vi "ReshapeItemArray.vi"(11 "Array":refnum<class "Link.lvclass">[](array[class])) -> (1 "ring info":refnum<class "RingItem.lvclass">[](array[class]), 3 "item info array":T1(array[cluster]))   [LabVIEW 2023, in "GettingStartedWindow.lvlib"]
uses:
  <resource>/modes/FRC/GettingStartedWindow.lvlib
  <resource>/modes/FRC/Classes/Link/Link.lvclass
  <resource>/modes/FRC/Classes/ClickableText/ClickableText.lvclass
  <resource>/modes/FRC/Classes/RingItem/RingItem.lvclass
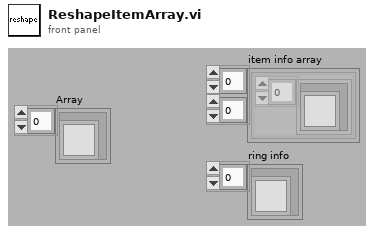
[diagram p1: front panel]
types:
  T1 = cluster{refnum<class "ClickableText.lvclass">[]}[][]
  T2 = typedef "GettingStartedWindow.lvlib/PositionCategory.ctl" = enum16{"none", "column 1", "column 2", "ring"}
  T3 = cluster{refnum<class "ClickableText.lvclass">[]}[]
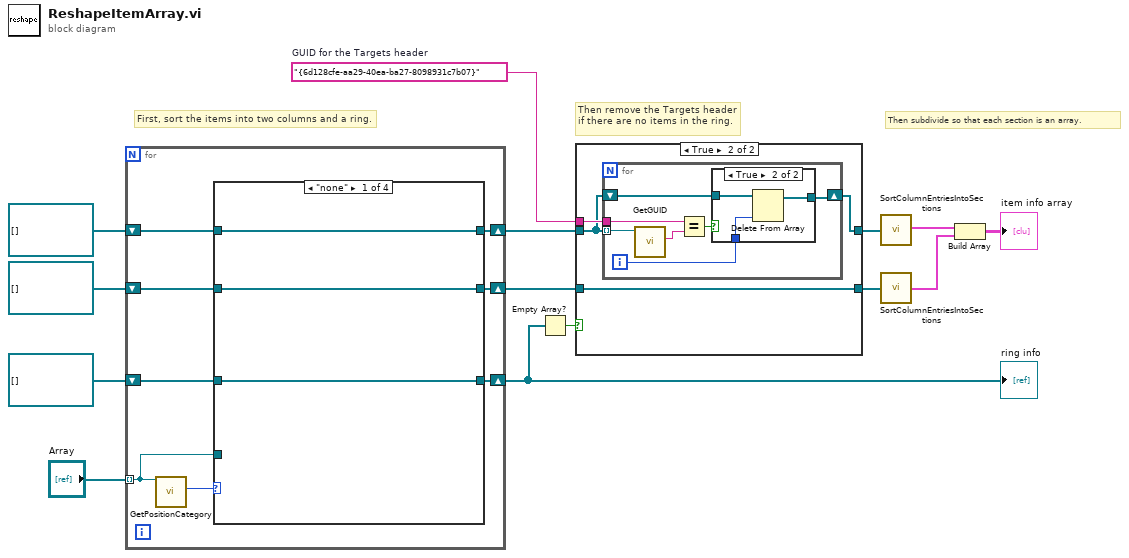
[diagram p0: block diagram]
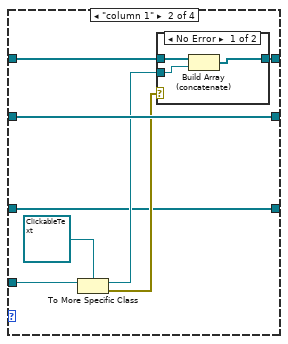
[diagram p4: hidden frame]
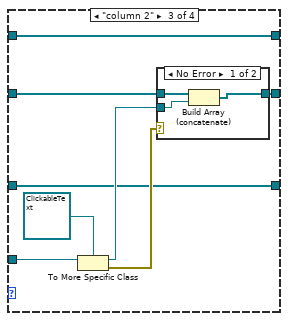
[diagram p6: hidden frame]
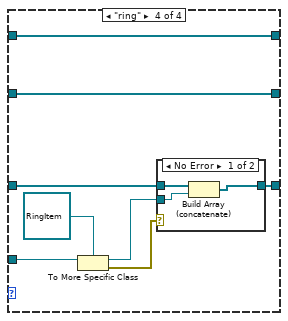
[diagram p8: hidden frame]
diagram:
  w1 = "{6d128cfe-aa29-40ea-ba27-8098931c7b07}"  # GUID for the Targets header
  # "Then remove the Targets header\nif there are no items in the ring."
  # "Then subdivide so that each section is an array."
  # "First, sort the items into two columns and a ring."
  n1 = for {
    tunnel: "Array" -> [w17] mode=indexing
    shift-right: [w20] -> w5
    shift-left: refnum<class "ClickableText.lvclass">[] [] -> [w21]
    shift-right: [w18] -> w3
    shift-left: refnum<class "ClickableText.lvclass">[] [] -> [w19]
    shift-right: [w15] -> w7
    shift-left: refnum<class "RingItem.lvclass">[] [] -> [w16]
    n2 = call-dynamic "GetPositionCategory.vi"("Link in"=w17) -> ("position"=w22:T2)  [unwired: 8 in, 2 out]
    n3 = case shown="\"none\"" w22 {
      tunnel: w21 -> [w25 w33 w40 w53]
      tunnel: w17 -> [_ w30 w45 w57]
      tunnel: [w25 w32 w40 w53] -> w20
      tunnel: w19 -> [w24 w31 w41 w52]
      tunnel: [w24 w31 w39 w52] -> w18
      tunnel: w16 -> [w23 w26 w38 w51]
      tunnel: [w23 w26 w38 w50] -> w15
      frame "none" {
      }
      frame "column 1" {
        n4 = To More Specific Class(target class=refnum<class "ClickableText.lvclass"> refnum ("GettingStartedWindow.lvlib:ClickableText.lvclass"), reference=w30) -> (specific class reference=w28:refnum<class "ClickableText.lvclass">, error out=w27:errorcluster)  [unwired: 1 in]
        n5 = case shown="No Error" w27 {
          tunnel: w33 -> [w36 w37]
          tunnel: [w35 w37] -> w32
          tunnel: w28 -> [w34 _]
          frame No Error {
            n6 = Build Array (concatenate)(w36, w34) -> (w35:refnum<class "ClickableText.lvclass">[])
          }
          frame Error {
          }
        }
      }
      frame "column 2" {
        n7 = To More Specific Class(target class=refnum<class "ClickableText.lvclass"> refnum ("GettingStartedWindow.lvlib:ClickableText.lvclass"), reference=w45) -> (specific class reference=w43:refnum<class "ClickableText.lvclass">, error out=w42:errorcluster)  [unwired: 1 in]
        n8 = case shown="No Error" w42 {
          tunnel: w41 -> [w48 w49]
          tunnel: [w47 w49] -> w39
          tunnel: w43 -> [w46 _]
          frame No Error {
            n9 = Build Array (concatenate)(w48, w46) -> (w47:refnum<class "ClickableText.lvclass">[])
          }
          frame Error {
          }
        }
      }
      frame "ring" {
        n10 = To More Specific Class(target class=refnum<class "RingItem.lvclass"> refnum ("GettingStartedWindow.lvlib:RingItem.lvclass"), reference=w57) -> (specific class reference=w55:refnum<class "RingItem.lvclass">, error out=w54:errorcluster)  [unwired: 1 in]
        n11 = case shown="No Error" w54 {
          tunnel: w51 -> [w60 w61]
          tunnel: [w59 w61] -> w50
          tunnel: w55 -> [w58 _]
          frame No Error {
            n12 = Build Array (concatenate)(w60, w58) -> (w59:refnum<class "RingItem.lvclass">[])
          }
          frame Error {
          }
        }
      }
    }
  }
  "ring info" <- w7
  n13 = Empty Array?(array=w7) -> (empty?=w6:bool)
  n14 = case shown="True" w6 {
    tunnel: w5 -> [w63 w65]
    tunnel: [w63 w64] -> w4
    tunnel: [w62 w67] -> w2
    tunnel: w3 -> [w62 w67]
    tunnel: w1 -> [_ w66]
    frame False {
    }
    frame True {
      n15 = for {
        tunnel: w65 -> [w74] mode=indexing
        tunnel: w66 -> [w72]
        shift-right: [w68] -> w64
        shift-left: w65 -> [w70]
        i -> [w69]
        n16 = call <resource>:"GetGUID.vi"("Link in"=w74) -> ("GUID"=w73:string)  [unwired: 8 in, 2 out]
        n17 = Equal?(x=w72, y=w73) -> (x = y?=w71:bool)
        n18 = case shown="True" w71 {
          tunnel: w70 -> [w75 w78]
          tunnel: w69 -> [_ w77]
          tunnel: [w75 w76] -> w68
          frame False {
          }
          frame True {
            n19 = Delete From Array(array=w78, index=w77) -> (array with subset deleted=w76:refnum<class "ClickableText.lvclass">[])  [unwired: 1 in, 1 out]
          }
        }
      }
    }
  }
  n20 = call <resource>:"SortColumnEntriesIntoSections.vi"("Array"=w4) -> ("Sorted Array"=w10:T3)
  n21 = call <resource>:"SortColumnEntriesIntoSections.vi"("Array"=w2) -> ("Sorted Array"=w8:T3)
  n22 = Build Array(w10, w8) -> (→"item info array":T1)
